vi "thermal_optical_capture_16.vi"() -> ()   [LabVIEW 2025]
uses:
  VIs_needed/Grab Manager Mode.ctl
  <vilib>/vision/driver/IMAQdx.llb/IMAQdx Buffer Number Mode.ctl
  <vilib>/vision/driver/NI_Vision_Acquisition_Software.lvlib
  <resource>/objmgr/imaqdx.rc
panel:
  in  "Stop":bool
  out "Images Saved Per Second":dbl
  out "Images Behind":i32
  out "Images Acquired Per Second":dbl
  in  "Skip Count":u32
  out "Write Speed Waveform":dbl(graph) caption="Image File Write Speed"
  out "Times between Frames":u32
  in  "Number of Images":u32=30
  in  "Camera Name":refnum<k21> caption="IMAQdx Session"
  out "Thermal Preview":T1(plugin-control)
  in  "Stop Preview":bool
  out "Times bw Thermal Frames":u32
  in  "STOP ACQUISITION":bool
  in  "Focus":dbl(slide) scale=0.0..100.0
  out "Thermal Frame Out":string
  in  "Output Folder":path
  in  "thermal capture interval (s)":dbl
  in  "Flag Button":bool
  in  "Stop & Save":bool
  in  "Record":bool
  # "Thermal Record"
  # "(Enter \"28\")"
  # "^ append to base data folder \"...\\test_n\\raw\" for nth recording"
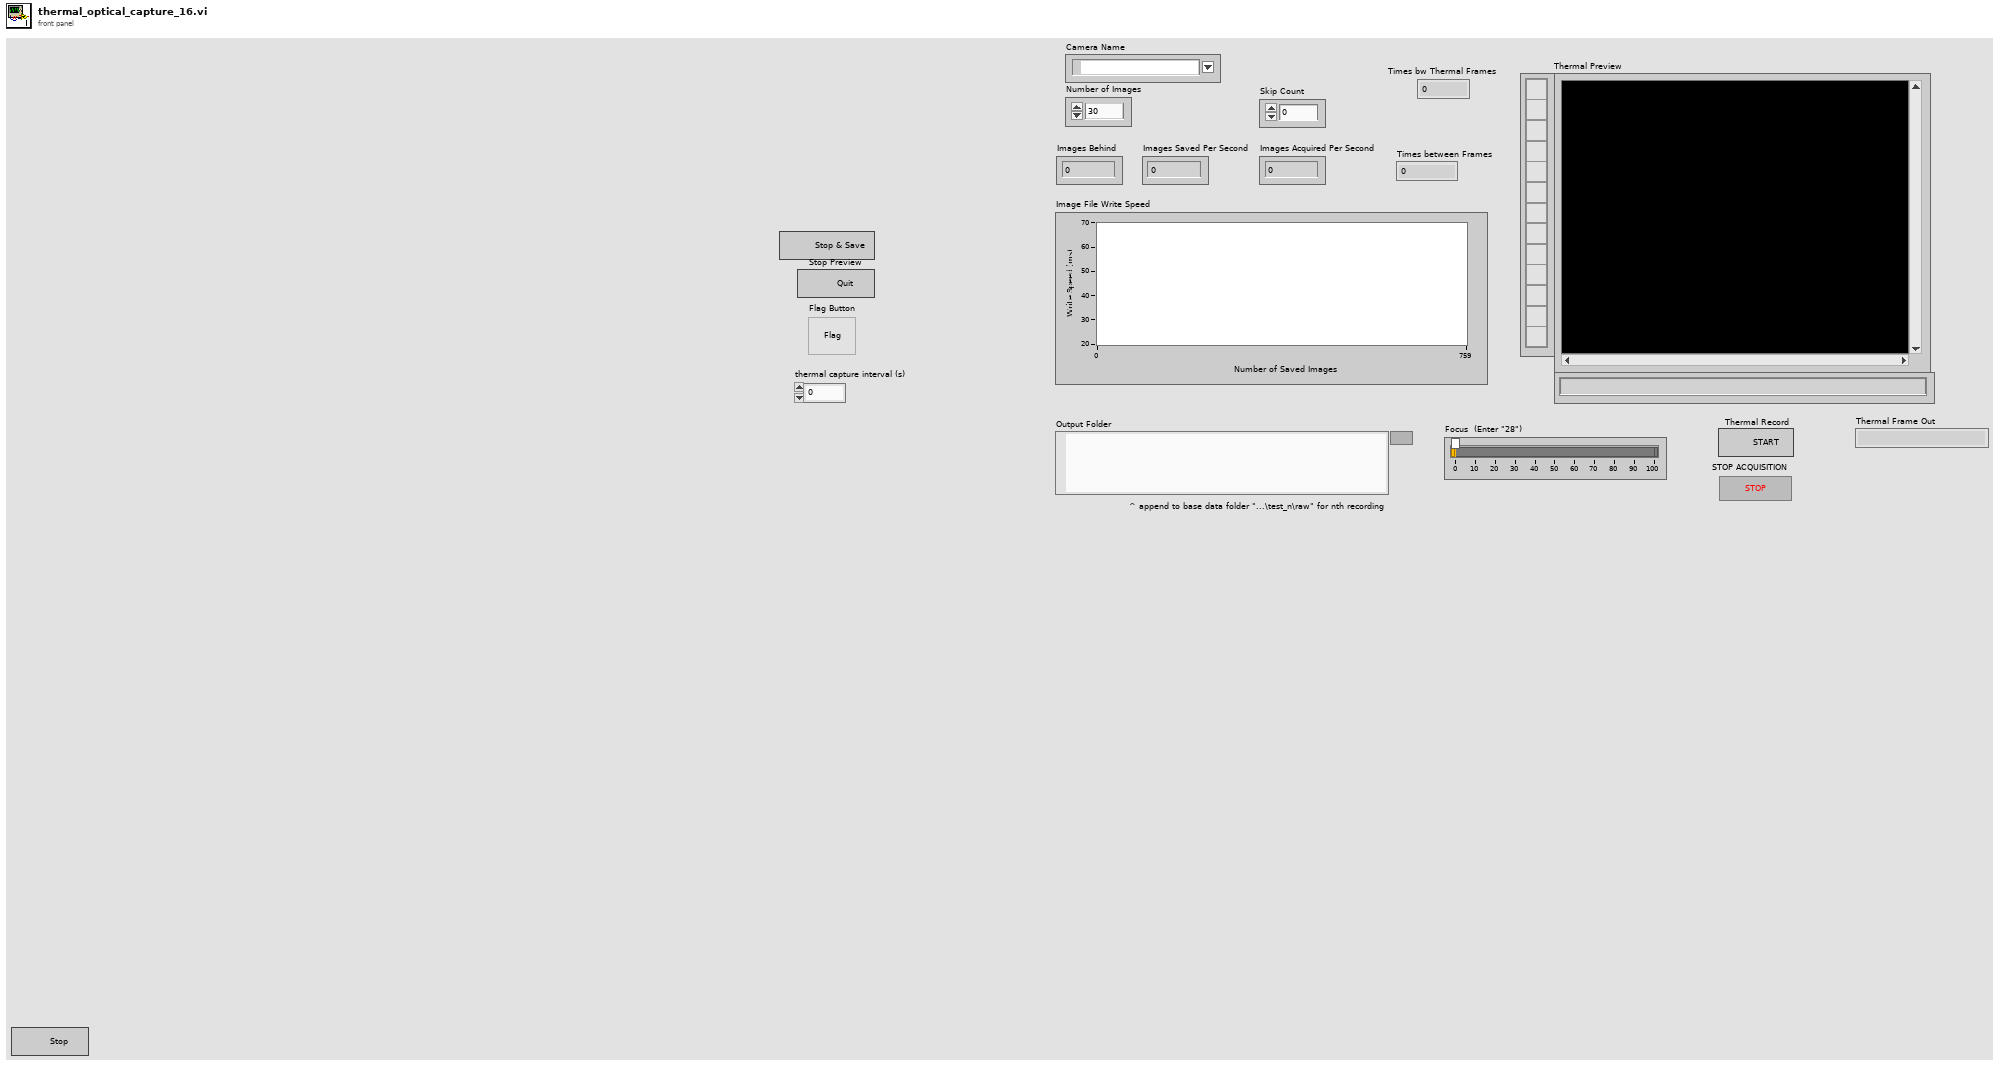
[diagram p1: front panel]
types:
  T1 = typedef "IMAQ Image.ctl" = refnum<image>
  T2 = typedef "Grab Manager Mode.ctl" = enum16{"Create Processing Images", "Lock", "Add Acquired Image", "Get Acquired Image", "Unlock", "Dispose Processing Images"}
  T3 = cluster{"Number of Processing Images":u32, "Image Border Size":u32}
  T4 = typedef "NI_Vision_Acquisition_Software.lvlib/IMAQdx Buffer Number Mode.ctl" = enum32{"Next", "Last", "Buffer Number", "Every", "Last New"}
  T5 = enum16{"open", "replace", "create", "open or create", "replace or create", "replace or create with confirmation"}
  T6 = enum16{"big-endian, network order", "native, host order", "little-endian"}
  T7 = typedef "Image Type" = u32
  T8 = typedef "IMAQdx.ctl" = refnum<k21>
  T9 = enum16{"Standard", "Buffered", "CRLF", "Immediate"}
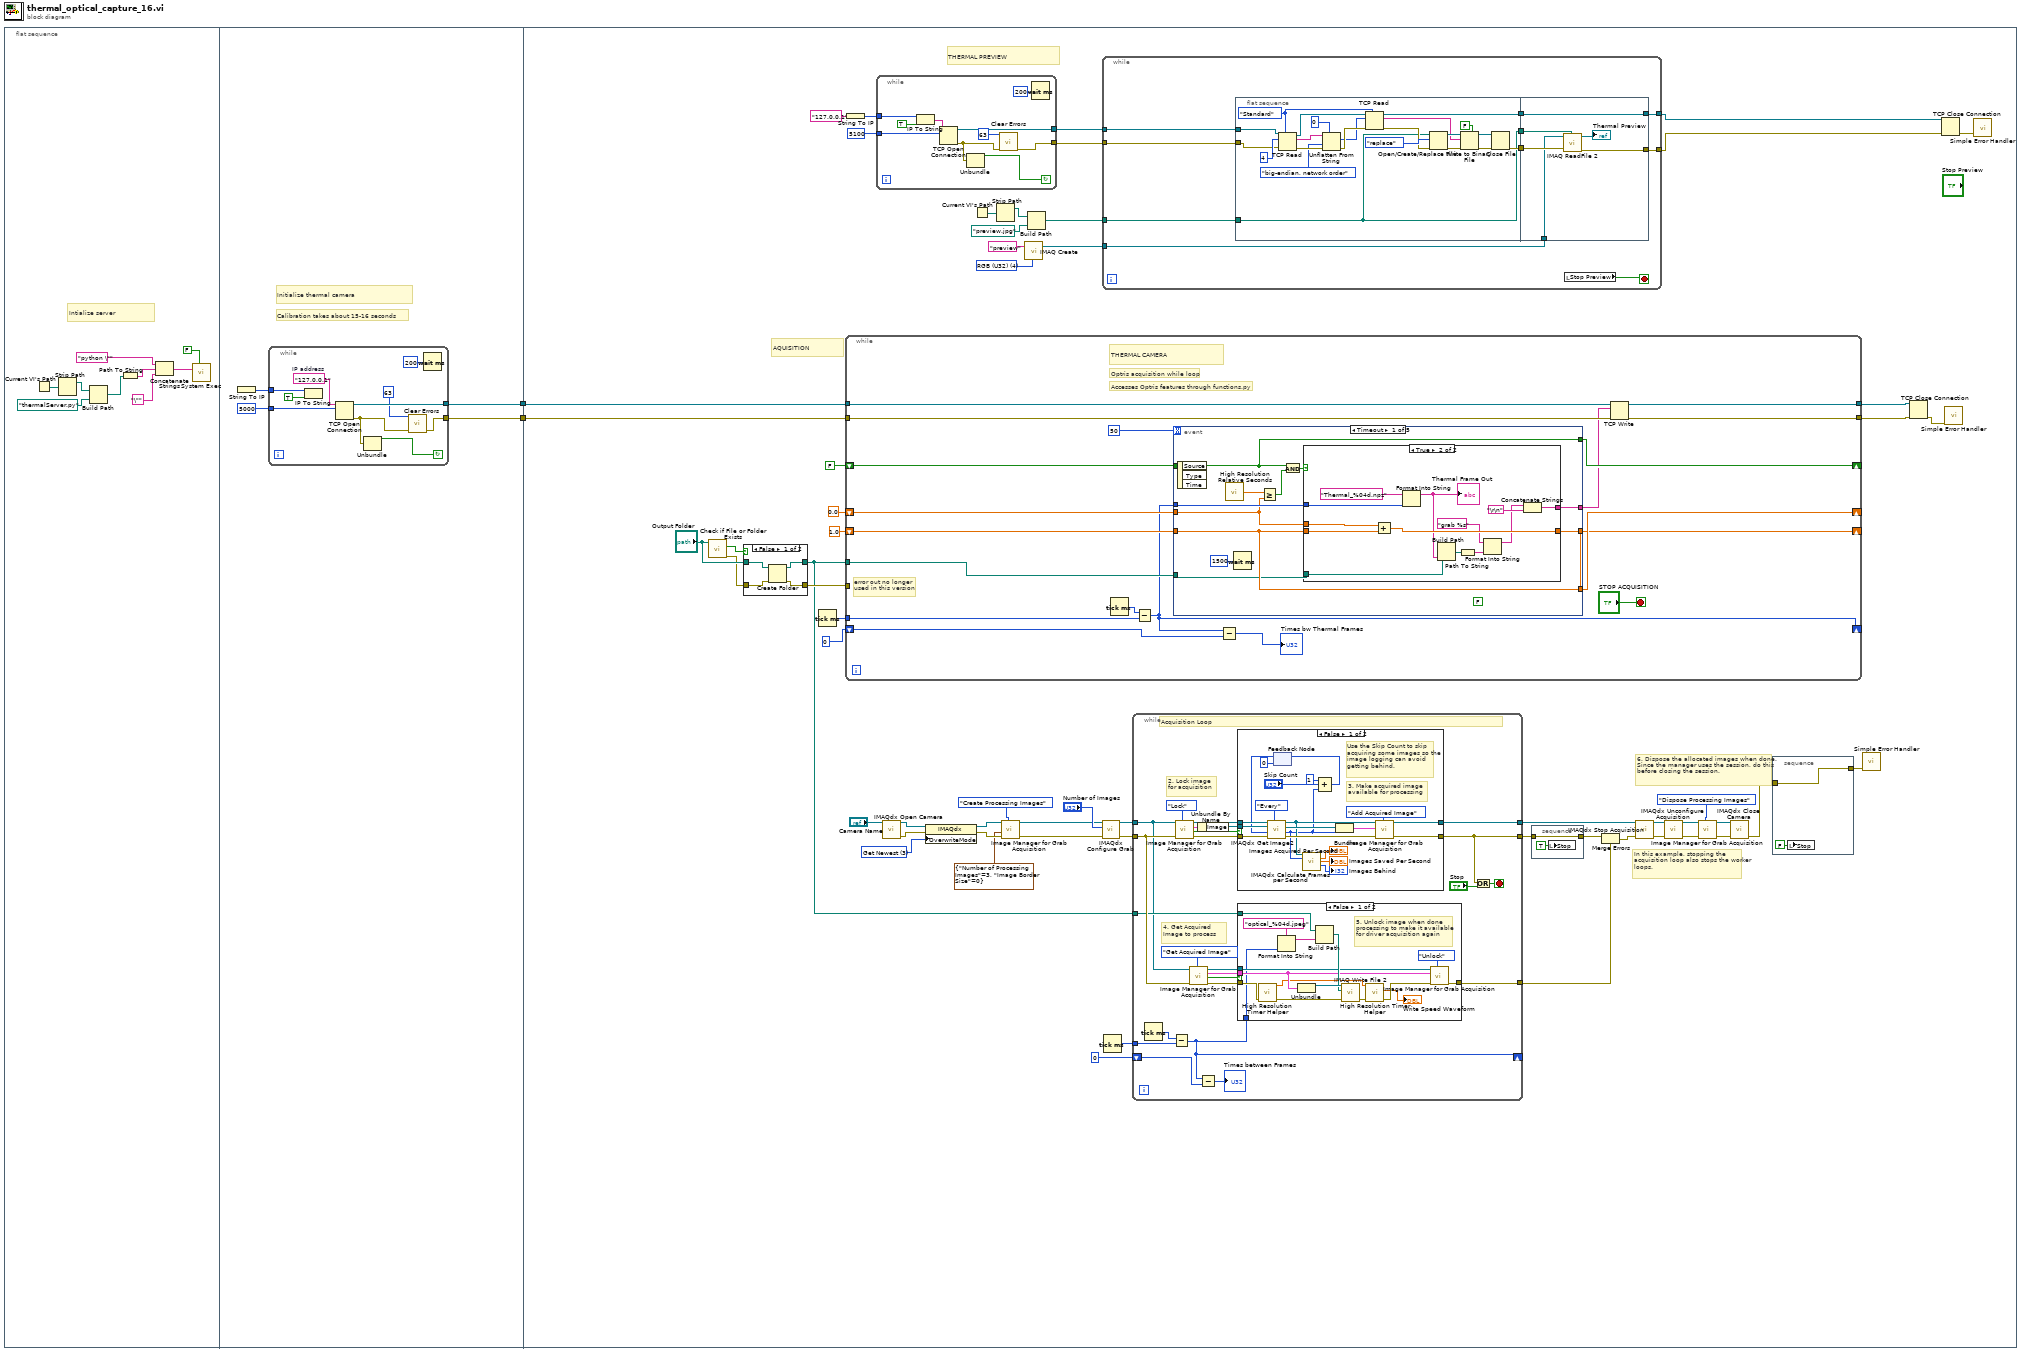
[diagram p0: block diagram]
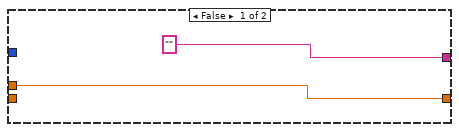
[diagram p5: hidden frame]
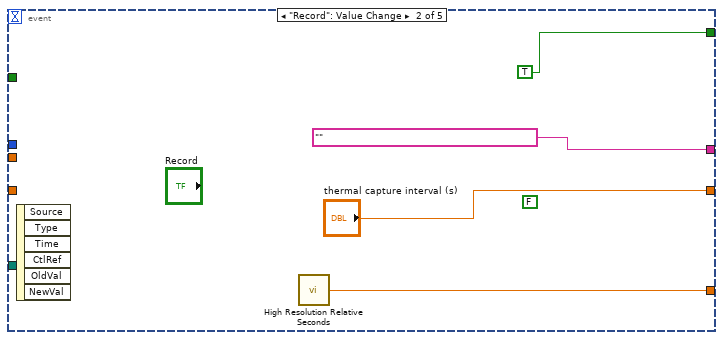
[diagram p6: hidden frame]
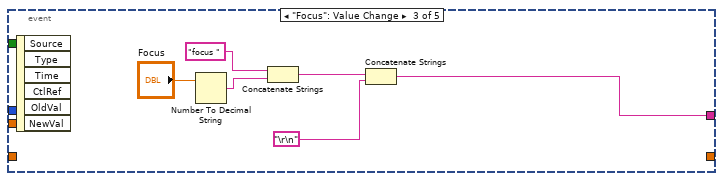
[diagram p7: hidden frame]
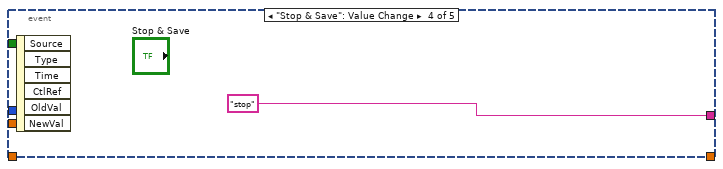
[diagram p8: hidden frame]
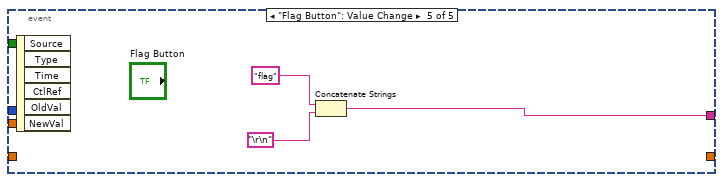
[diagram p9: hidden frame]
diagram:
  n1 = flat-sequence {
    tunnel: [w13] -> w2
    tunnel: [w12] -> w1
    tunnel: w1 -> [w81]
    tunnel: w2 -> [w80]
    frame #0 {
      # "Intialize server"
      n2 = Current VI's Path() -> (path=w6:path)
      n3 = Strip Path(path=w6) -> (stripped path=w7:path)  [unwired: 1 out]
      n4 = Build Path(base path=w7, name or relative path=path "thermalServer.py") -> (appended path=w4:path)
      n5 = Path To String(path=w4) -> (string=w10:string)
      n6 = Concatenate Strings("python \"" ("string"), w10, "\"" ("string")) -> (w9:string)
      n7 = call <vilib>:"System Exec.vi"("wait until completion? (T)"=FALSE, "command line"=w9) -> ()  [unwired: 6 in, 4 out]
    }
    frame #1 {
      # "Initialize thermal camera"
      # "Calibration takes about 15-16 seconds"
      n8 = String To IP() -> (0:w15:u32)  [unwired: 1 in]
      n9 = while {
        tunnel: [w20] -> w13
        tunnel: [w25] -> w12
        tunnel: w15 -> [w24]
        tunnel: u16 5000 ("remote port or service name") -> [w22]
        stop <- w17 continue-if-true
        w16 = "127.0.0.1"  # IP address
        n10 = IP To String(1:TRUE ("dot notation? (F)"), 2:w24) -> ()  [unwired: 1 out]
        n11 = TCP Open Connection(address=w16, remote port or service name=w22) -> (connection ID=w25:refnum<k5>, error out=w21:errorcluster)  [unwired: 3 in]
        n12 = Unbundle(w21) -> ("status"=w17:bool)  [unwired: 2 out]
        n13 = call <vilib>:"Clear Errors.vi"("error in (no error)"=w21, "specific error code to clear (0: all)"=63) -> ("error out"=w20:errorcluster)  [unwired: 4 in, 1 out]
        n14 = Wait (ms)(milliseconds to wait=u32 200) -> ()  [unwired: 1 out]
      }
    }
    frame #2 {
      w28 = u32 3 items=["Get Oldest"=0, "Fail"=2, "Get Newest"=3] ("OverwriteMode")
      w68 = T7 4 items=["Grayscale (U8)", "Grayscale (I16)", "Grayscale (SGL)", "Complex (CSG)", "RGB (U32)", "HSL (U32)", "RGB (U64)", "Grayscale (U16)"] ("Image Type")
      # "6. Dispose the allocated images when done. Since the manager uses the session, do this before closing the session."
      # "In this example, stopping the acquisition loop also stops the worker loops."
      # "THERMAL PREVIEW"
      # "AQUISITION"
      n15 = call <vilib>:"Check if File or Folder Exists.vi"("path"="Output Folder") -> ("error out"=w60:errorcluster, "file or folder exists?"=w62:bool)  [unwired: 8 in, 1 out]
      n16 = case shown="False" w62 {
        tunnel: "Output Folder" -> [w155 w157]
        tunnel: [w154 w157] -> w55
        tunnel: w60 -> [w153 w156]
        tunnel: [w152 w156] -> w59
        frame False {
          n17 = Create Folder(path (use dialog)=w155, error in=w153) -> (created path=w154:path, error out=w152:errorcluster)  [unwired: 1 in, 1 out]
        }
        frame True {
        }
      }
      n18 = Tick Count (ms)() -> (millisecond timer value=w76:u32)
      n19 = while {
        tunnel: [w224] -> w82
        tunnel: [w223] -> w83
        tunnel: w81 -> [w222]
        tunnel: w80 -> [w221]
        shift-right: [w220] -> _
        shift-left: 0.0 -> [w217]
        shift-right: [w218] -> _
        shift-left: 1.0 -> [w215]
        shift-right: [w219] -> _
        shift-left: FALSE -> [w216]
        tunnel: w76 -> [w214]
        shift-right: [w211] -> _
        shift-left: u32 0 -> [w213]
        tunnel: w55 -> [w212]
        tunnel: w59 -> [_]
        stop <- "STOP ACQUISITION" stop-if-true
        # "error out no longer used in this version"
        # "THERMAL CAMERA"
        # "Optris acquisition while loop"
        # "Accesses Optris features through functions.py"
        n20 = Tick Count (ms)() -> (millisecond timer value=w207:u32)
        n21 = Subtract(x=w207, y=w214) -> (x-y=w211:u32)
        n22 = event shown="[0] Timeout" {
          selector: _ -> [_ _ _ _ _]
          dyn-events: _ -> [_ _ _ _ _]
          timeout: 50 -> [_ _ _ _ _]
          tunnel: [w231 "" w255 "stop" w264] -> w208
          tunnel: w211 -> [w232 _ _ _ _]
          tunnel: [w229 w254 _ _ _] -> w220
          tunnel: [w227 TRUE _ _ _] -> w219
          tunnel: [w228 "thermal capture interval (s)" _ _ _] -> w218
          tunnel: w217 -> [w230 _ _ _ _]
          tunnel: w216 -> [w227 _ _ _ _]
          tunnel: w215 -> [w228 _ _ _ _]
          tunnel: w212 -> [w226 _ _ _ _]
          event Timeout {
            (unwired) FALSE
            n23 = event-data() -> ()  [unwired: 1 in, 3 out]
            n24 = call <vilib>:"High Resolution Relative Seconds.vi"() -> ("relative seconds"=w235:dbl)
            n25 = Wait (ms)(milliseconds to wait=u32 1500) -> ()  [unwired: 1 out]
            n26 = Greater Or Equal?(x=w235, y=w230) -> (x >= y?=w234:bool)
            n27 = And(x=w227, y=w234) -> (x .and. y?=w233:bool)
            n28 = case shown="True" w233 {
              tunnel: w232 -> [_ w248]
              tunnel: ["" w249] -> w231
              tunnel: w230 -> [w236 w247]
              tunnel: w228 -> [_ w246]
              tunnel: [w236 w245] -> w229
              tunnel: w226 -> [_ w238]
              frame False {
              }
              frame True {
                n29 = Add(x=w247, y=w246) -> (x+y=w245:dbl)
                n30 = Format Into String(format string="Thermal_%04d.npz", w248) -> (resulting string=w239:string)  [unwired: 2 in, 1 out]
                "Thermal Frame Out" <- w239
                n31 = Build Path(base path=w238, name or relative path=w239) -> (appended path=w243:path)
                n32 = Path To String(path=w243) -> (string=w241:string)
                n33 = Format Into String(format string="grab %s", w241) -> (resulting string=w240:string)  [unwired: 2 in, 1 out]
                n34 = Concatenate Strings(w240, "\r\n") -> (w249:string)
              }
            }
          }
          event "Record": Value Change {
            (unwired) FALSE
            n35 = event-data() -> ()  [unwired: 1 in, 6 out]
            n36 = call <vilib>:"High Resolution Relative Seconds.vi"() -> ("relative seconds"=w254:dbl)
          }
          event "Focus": Value Change {
            n37 = event-data() -> ()  [unwired: 1 in, 6 out]
            n38 = Number To Decimal String(number="Focus") -> (decimal integer string=w260:string)  [unwired: 1 in]
            n39 = Concatenate Strings("focus ", w260) -> (w257:string)
            n40 = Concatenate Strings(w257, "\r\n") -> (w255:string)
          }
          event "Stop & Save": Value Change {
            n41 = event-data() -> ()  [unwired: 1 in, 6 out]
          }
          event "Flag Button": Value Change {
            n42 = event-data() -> ()  [unwired: 1 in, 6 out]
            n43 = Concatenate Strings("flag", "\r\n") -> (w264:string)
          }
        }
        n44 = Subtract(x=w211, y=w213) -> (x-y=→"Times bw Thermal Frames":u32)
        n45 = TCP Write(connection ID=w222, data in=w208, error in (no error)=w221) -> (connection ID out=w223:refnum<k5>, error out=w224:errorcluster)  [unwired: 1 in, 1 out]
      }
      n46 = String To IP(1:"127.0.0.1" ("name")) -> (0:w67:u32)
      n47 = while {
        tunnel: w67 -> [w167]
        tunnel: [w161] -> w66
        tunnel: [w165] -> w65
        tunnel: u16 5100 ("remote port or service name") -> [w163]
        stop <- w158 continue-if-true
        n48 = IP To String(1:TRUE ("dot notation? (F)"), 2:w167) -> (0:w166:string)
        n49 = TCP Open Connection(address=w166, remote port or service name=w163) -> (connection ID=w165:refnum<k5>, error out=w162:errorcluster)  [unwired: 3 in]
        n50 = Unbundle(w162) -> ("status"=w158:bool)  [unwired: 2 out]
        n51 = call <vilib>:"Clear Errors.vi"("error in (no error)"=w162, "specific error code to clear (0: all)"=63) -> ("error out"=w161:errorcluster)  [unwired: 4 in, 1 out]
        n52 = Wait (ms)(milliseconds to wait=u32 200) -> ()  [unwired: 1 out]
      }
      n53 = call <vilib>:"IMAQdx Open Camera.vi"("Session In"="Camera Name") -> ("error out"=w50:errorcluster, "Session Out"=w51:T8)  [unwired: 2 in, 7 out]
      n54 = property class="IMAQdx"(reference=w51, error in=w50, "OverwriteMode"=w28) -> (reference out=w53:T8, error out=w52:errorcluster)
      n55 = Current VI's Path() -> (path=w73:path)
      n56 = Strip Path(path=w73) -> (stripped path=w74:path)  [unwired: 1 out]
      n57 = call "Image Manager for Grab Acquisition.vi"("Mode"=Grab_Manager_Mode."Create Processing Images", "error in (no error)"=w52, "Init Settings"=T3 {"Number of Processing Images"=3, "Image Border Size"=0}, "Session In"=w53) -> ("error out"=w48:errorcluster, "Session Out"=w47:T8)  [unwired: 4 in, 2 out]
      n58 = call "IMAQ Create"("Image Name"="preview", "Image Type"=w68) -> ("New Image"=w71:T1)  [unwired: 3 in, 1 out]
      n59 = Build Path(base path=w74, name or relative path=path "preview.jpg") -> (appended path=w72:path)
      n60 = while {
        tunnel: w71 -> [w172]
        tunnel: [w173] -> w57
        tunnel: [w177] -> w56
        tunnel: w72 -> [w175]
        tunnel: w66 -> [w170]
        tunnel: w65 -> [w169]
        stop <- w168 stop-if-true
        n61 = flat-sequence {
          tunnel: w175 -> [w181]
          tunnel: [w183] -> w176
          tunnel: [w182] -> w174
          tunnel: [w181] -> w171
          tunnel: w170 -> [w179]
          tunnel: w169 -> [w178]
          tunnel: [w205] -> w177
          tunnel: w176 -> [w205]
          tunnel: w174 -> [w204]
          tunnel: [w203] -> w173
          tunnel: w172 -> [w202]
          tunnel: w171 -> [w201]
          frame #0 {
            w192 = T9."Standard" ("mode (standard)")
            n62 = TCP Read(connection ID=w178, bytes to read=4, error in (no error)=w179, 7:w192) -> (connection ID out=w195:refnum<k5>, data out=w180:string, error out=w198:errorcluster)  [unwired: 1 in]
            n63 = Unflatten From String(type=0, binary string=w180, byte order (0:big-endian, network order)=T6."big-endian, network order", error in (no error)=w198) -> (value=w193:i32, error out=w194:errorcluster)  [unwired: 1 in, 1 out]
            n64 = TCP Read(connection ID=w195, bytes to read=w193, error in (no error)=w194, 7:w192) -> (connection ID out=w183:refnum<k5>, data out=w188:string, error out=w190:errorcluster)  [unwired: 1 in]
            n65 = Open/Create/Replace File(file path (use dialog)=w181, error in=w190, operation (0:open)=T5."replace") -> (refnum out=w189:refnum<file>, error out=w186:errorcluster)  [unwired: 3 in, 1 out]
            n66 = Write to Binary File(file (use dialog)=w189, data=w188, error in=w186, 5:FALSE ("prepend array or string size? (T)")) -> (refnum out=w184:refnum<file>, error out=w185:errorcluster)  [unwired: 2 in, 1 out]
            n67 = Close File(refnum=w184, error in=w185) -> (error out=w182:errorcluster)  [unwired: 1 out]
          }
          frame #1 {
            n68 = call "IMAQ ReadFile 2"("File Path"=w201, "error in (no error)"=w204, "Image"=w202) -> ("error out"=w203:errorcluster, "Image Out"=→"Thermal Preview":T1)  [unwired: 4 in, 3 out]
          }
        }
        n69 = local read "Stop Preview"() -> (w168:bool)
      }
      n70 = call <vilib>:"IMAQdx Configure Grab.vi"("error in"=w48, "Number of Buffers"="Number of Images", "Session In"=w47) -> ("error out"=w32:errorcluster, "Session Out"=w33:T8)  [unwired: 7 in]
      n71 = Tick Count (ms)() -> (millisecond timer value=w31:u32)
      n72 = while {
        tunnel: w32 -> [w102]
        tunnel: w33 -> [w100]
        tunnel: [w109] -> w43
        tunnel: [w110] -> w42
        tunnel: w55 -> [w101]
        tunnel: [w99] -> w34
        tunnel: w31 -> [w92]
        shift-right: [w89] -> _
        shift-left: u32 0 -> [w90]
        stop <- w111 stop-if-true
        # "4. Get Acquired Image to process"
        # "2. Lock image for acquisition"
        # "Acquisition Loop"
        n73 = Tick Count (ms)() -> (millisecond timer value=w93:u32)
        n74 = Subtract(x=w93, y=w92) -> (x-y=w89:u32)
        n75 = call "Image Manager for Grab Acquisition.vi"("Mode"=Grab_Manager_Mode."Lock", "error in (no error)"=w102, "Session In"=w100) -> ("error out"=w105:errorcluster, "No Available Image"=w106:bool, "Image Settings Out"=w104:cluster{"Image":T1, "Buffer Number":u32}, "Session Out"=w107:T8)  [unwired: 5 in]
        n76 = call "Image Manager for Grab Acquisition.vi"("Mode"=Grab_Manager_Mode."Get Acquired Image", "error in (no error)"=w102, "Session In"=w100) -> ("error out"=w95:errorcluster, "No Available Image"=w97:bool, "Image Settings Out"=w96:cluster{"Image":T1, "Buffer Number":u32}, "Session Out"=w94:T8)  [unwired: 5 in]
        n77 = Unbundle By Name(w104) -> ("Image"=w103:T1)
        n78 = Subtract(x=w89, y=w90) -> (x-y=→"Times between Frames":u32)
        n79 = case shown="False" w106 {
          tunnel: [w141 w151] -> w109
          tunnel: [w140 w150] -> w110
          tunnel: w107 -> [w149 w151]
          tunnel: w105 -> [w148 w150]
          tunnel: w103 -> [w142 _]
          frame False {
            # "3. Make acquired image available for processing"
            # "Use the Skip Count to skip acquiring some images so the image logging can avoid getting behind."
            n80 = feedback #1(u32 0) -> (w131:u32)
            n81 = call <vilib>:"IMAQdx Get Image2.vi"("Buffer Number Mode (Next)"=IMAQdx_Buffer_Number_Mode."Every", "error in"=w148, "Buffer Number In"=w131, "Image In"=w142, "Session In"=w149) -> ("error out"=w144:errorcluster, "Buffer Number Out"=w135:u32, "Image Out"=w146:T1, "Session Out"=w139:T8)  [unwired: 3 in]
            n82 = call <vilib>:"IMAQdx Calculate Frames per Second.vi"("Session In"=w139, "Buffer Number"=w135) -> ("Acquired Frames per Second"=→"Images Acquired Per Second":dbl, "Processed Frames per Second"=→"Images Saved Per Second":dbl, "Images Behind"=→"Images Behind":i32)  [unwired: 7 in, 4 out]
            n83 = Compound Arithmetic op=ADD(u32 1 ("value"), "Skip Count", w135) -> (w132:u32)
            n84 = feedback-in #1(w132) -> ()
            n85 = Bundle("Image Out"=w146, "Buffer Number Out"=w135) -> (w145:cluster{"Image Out":T1, "Buffer Number Out":u32})  [unwired: 1 in]
            n86 = call "Image Manager for Grab Acquisition.vi"("Mode"=Grab_Manager_Mode."Add Acquired Image", "error in (no error)"=w144, "Image Settings In"=w145, "Session In"=w139) -> ("error out"=w140:errorcluster, "Session Out"=w141:T8)  [unwired: 4 in, 2 out]
          }
          frame True {
            # "The Lock function already has a delay inside when no images are available to prevent loop from going too fast and starving the worker threads from getting processing time."
            # "Write to disk operation is taking longer so images aren't added back to manager. Wait until there is an available image"
          }
        }
        n87 = case shown="False" w97 {
          tunnel: w95 -> [w119 w129]
          tunnel: w96 -> [w121 _]
          tunnel: [w123 w129] -> w99
          tunnel: w101 -> [w127 _]
          tunnel: w94 -> [w120 _]
          tunnel: w89 -> [w113 _]
          frame False {
            # "5. Unlock image when done processing to make it available for driver acquisition again"
            n88 = call "High Resolution Timer Helper.vi"("error in (no error)"=w119) -> ("error out"=w118:errorcluster, "Current Time"=w114:dbl)  [unwired: 8 in, 1 out]
            n89 = Format Into String(format string="optical_%04d.jpeg", w113) -> (resulting string=w126:string)  [unwired: 2 in, 1 out]
            n90 = Unbundle(w121) -> ("Image"=w128:T1)  [unwired: 1 out]
            n91 = Build Path(base path=w127, name or relative path=w126) -> (appended path=w124:path)
            n92 = call-poly "IMAQ Write File 2"("error in (no error)"=w118, "File Path"=w124, "Image"=w128) -> ("error out"=w117:errorcluster)  [unwired: 7 in, 1 out]
            n93 = call "High Resolution Timer Helper.vi"("error in (no error)"=w117, "Previous Time"=w114) -> ("error out"=w116:errorcluster, "Time Difference (ms)"=→"Write Speed Waveform":dbl)  [unwired: 7 in, 1 out]
            n94 = call "Image Manager for Grab Acquisition.vi"("Mode"=Grab_Manager_Mode."Unlock", "error in (no error)"=w116, "Image Settings In"=w121, "Session In"=w120) -> ("error out"=w123:errorcluster)  [unwired: 4 in, 3 out]
          }
          frame True {
            # "No acquired images to process"
          }
        }
        n95 = Or(x=w110, y="Stop") -> (x .or. y?=w111:bool)
      }
      n96 = stacked-sequence {
        tunnel: [w87] -> w41
        tunnel: w42 -> [w87]
        frame #0 {
          n97 = local write "Stop"(TRUE ("Stop")) -> ()
        }
      }
      n98 = Merge Errors(w41, w34) -> (w44:errorcluster)
      n99 = call <vilib>:"IMAQdx Stop Acquisition.vi"("error in"=w44, "Session In"=w43) -> ("error out"=w45:errorcluster, "Session Out"=w46:T8)  [unwired: 8 out]
      n100 = call <vilib>:"IMAQdx Unconfigure Acquisition.vi"("error in"=w45, "Session In"=w46) -> ("error out"=w38:errorcluster, "Session Out"=w39:T8)  [unwired: 8 out]
      n101 = call "Image Manager for Grab Acquisition.vi"("Mode"=Grab_Manager_Mode."Dispose Processing Images", "error in (no error)"=w38, "Session In"=w39) -> ("error out"=w36:errorcluster, "Session Out"=w37:T8)  [unwired: 5 in, 2 out]
      n102 = call <vilib>:"IMAQdx Close Camera.vi"("error in"=w36, "Session In"=w37) -> ("error out"=w35:errorcluster)  [unwired: 9 out]
      n103 = stacked-sequence {
        tunnel: [w85] -> w40
        tunnel: w35 -> [w85]
        frame #0 {
          n104 = local write "Stop"(FALSE ("Stop")) -> ()
        }
      }
      n105 = call <vilib>:"Simple Error Handler.vi"("error in (no error)"=w40) -> ()  [unwired: 4 in, 5 out]
      n106 = TCP Close Connection(connection ID=w83, error in (no error)=w82) -> (error out=w84:errorcluster)  [unwired: 1 in, 1 out]
      n107 = TCP Close Connection(connection ID=w56, error in (no error)=w57) -> (error out=w58:errorcluster)  [unwired: 1 in, 1 out]
      n108 = call <vilib>:"Simple Error Handler.vi"("error in (no error)"=w84) -> ()  [unwired: 4 in, 5 out]
      n109 = call <vilib>:"Simple Error Handler.vi"("error in (no error)"=w58) -> ()  [unwired: 4 in, 5 out]
    }
  }
